vi "Handle Drag.vi"(7 "Done? (F)":bool, 9 "Available Data Names":string[](array[string]), 10 "Coords":T1, 11 "SequenceViewPanel in":refnum<class "SequenceViewPanel.lvclass">) -> (1 "Tag":string, 2 "Step Type Name":string, 3 "SequenceViewPanel out":refnum<class "SequenceViewPanel.lvclass">, 4 "Accepted?":bool, 5 "Index":i32)   [LabVIEW 2020, in "TSnax UI.lvlib" / "SequenceViewPanel.lvclass"]
uses:
  SequenceViewPanel.lvclass
  <vilib>/Utility/miscctls.llb/LVPoint32TypeDef.ctl
  Drag Data Names.ctl
  SequenceViewPanel.lvclass/SequenceViewPanel.ctl
  52703bb3-bc71-497d-a9d4-2f3dd9cc266b.vi
  11c460cf-3c17-418e-a9ab-802b58c45a96.vi
  ed1cb1d0-fc78-41af-bcfe-643c78fa2054.vi
  <vilib>/Comparison/Equal/Equal Functor/Equal Functor.lvclass
  TSnax UI.lvlib
panel:
  out "Top Index":i32
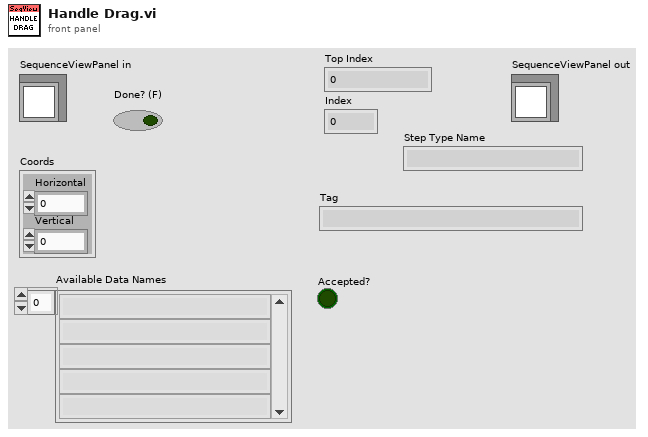
[diagram p1: front panel]
types:
  T1 = typedef "LVPoint32TypeDef.ctl" = cluster{"Horizontal":i32, "Vertical":i32}
  T2 = typedef "TSnax UI.lvlib/Drag Data Names.ctl" = enum16{"TSnax_InsertStep"}
  T3 = typedef "LVNodeAndColumnTypeDef.ctl" = cluster{"Node":string, "Column":i32}
  T4 = typedef "TSnax UI.lvlib/SequenceViewPanel.lvclass/Ref Data.ctl" = cluster{"Insert Line":i32, "SequenceFile":refnum<class "SequenceFile.lvclass">, "Sequence":string}
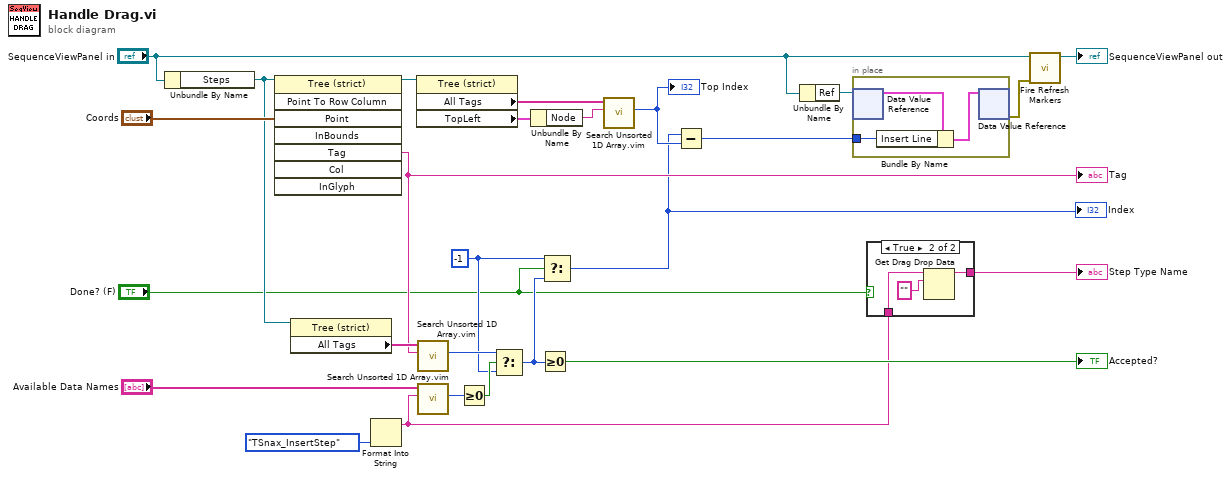
[diagram p0: block diagram]
diagram:
  w11 = -1 ("f")
  n1 = Unbundle By Name("SequenceViewPanel in") -> ("Steps"=w16:refnum<vi>)
  n2 = invoke on="Invoke Node" class="Tree (strict)" method="Point To Row Column"(reference=w16, "Point"="Coords") -> (reference out=w7:refnum<vi>, "Tag"=w25:string)  [unwired: 6 in, 6 out]
  "Tag" <- w25
  n3 = property on="Property Node" class="Tree (strict)"(reference=w16) -> ("All Tags"=w26:string[])  [unwired: 1 in, 2 out]
  n4 = Format Into String(Drag_Data_Names."TSnax_InsertStep" ("Drag Data Names")) -> (resulting string=w9:string)  [unwired: 3 in, 1 out]
  n5 = property class="Tree (strict)"(reference=w7) -> ("All Tags"=w5:string[], "TopLeft"=w6:T3)  [unwired: 1 in, 2 out]
  n6 = call "Search Unsorted 1D Array.vim"("element"=w25, "unsorted 1D array"=w26) -> ("index of element"=w21:i32)  [unwired: 9 in]
  n7 = call "Search Unsorted 1D Array.vim"("element"=w9, "unsorted 1D array"="Available Data Names") -> ("index of element"=w22:i32)  [unwired: 9 in]
  n8 = Greater Or Equal To 0?(x=w22) -> (x >= 0?=w20:bool)
  n9 = Select(t=w21, s=w20, f=w11) -> (s? t:f=w12:i32)
  n10 = Unbundle By Name(w6) -> ("Node"=w4:string)
  n11 = Greater Or Equal To 0?(x=w12) -> (x >= 0?=→"Accepted?":bool)
  n12 = Select(t=w11, s="Done? (F)", f=w12) -> (s? t:f=w2:i32)
  "Index" <- w2
  n13 = call "Search Unsorted 1D Array.vim"("element"=w4, "unsorted 1D array"=w5) -> ("index of element"=w3:i32)  [unwired: 9 in]
  "Top Index" <- w3
  n14 = Subtract(x=w2, y=w3) -> (x-y=w1:i32)
  n15 = Unbundle By Name("SequenceViewPanel in") -> ("Ref"=w24:refnum<data-value>)
  n16 = in-place {
    in-place-border: w1 -> [w27]
    n17 = in-place-dvr #1(w24) -> (w29:T4)  [unwired: 1 out]
    n18 = Bundle By Name(cluster=w29, "Insert Line"=w27) -> (w28:T4)
    n19 = in-place-dvr #1(w28) -> (w13:errorcluster)  [unwired: 1 out]
  }
  n20 = case shown="True" "Done? (F)" {
    tunnel: w9 -> [_ w31]
    tunnel: [_ w30] -> w8
    frame False {
    }
    frame True {
      n21 = Get Drag Drop Data(8:"", 9:w31) -> (3:w30:string)  [unwired: 1 in, 1 out]
    }
  }
  "Step Type Name" <- w8
  n22 = call "Fire Refresh Markers.vi"("error in (no error)"=w13, "SequenceViewPanel in"="SequenceViewPanel in") -> ("SequenceViewPanel out"=→"SequenceViewPanel out":refnum<class "SequenceViewPanel.lvclass">)  [unwired: 8 in, 1 out]
